vi "G#Debugger_Init.vi"(0 "This VI":refnum<vi>, 5 "error in (no error)":errorcluster) -> (14 "refs":T1, 16 "GUI Event Registration Refnum":refnum<event-registration>, 17 "Application Instance":string, 19 "error out":errorcluster)   [LabVIEW 2017, in "G#Debugger.lvlib"]
uses:
  G#Debugger.lvlib
  G#Debugger_Refs.ctl
  G#Object/utils/G#Object_ClassInfoType.ctl
  G#Object/G#Object.lvclass
  G#Object/utils/G#Object_ObjectInfoType.ctl
  G#Object/utils/G#Object_CreateMethod.ctl
  G#Debugger_SubPanelInfo.ctl
  G#Object/utils/G#Object_ClassHierarchy.ctl
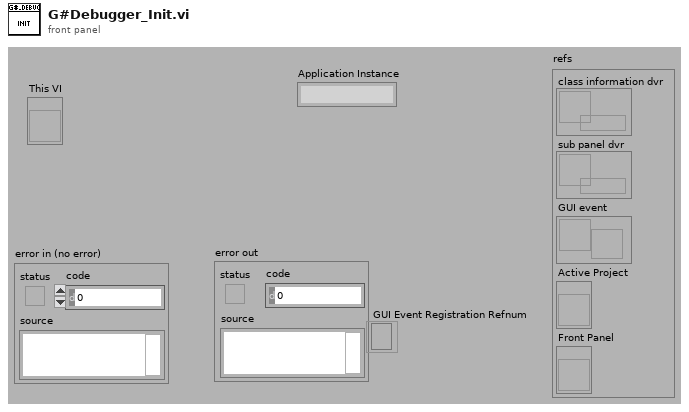
[diagram p1: front panel]
types:
  T1 = typedef "G#Debugger.lvlib/G#Debugger_Refs.ctl" = cluster{"class information dvr":refnum<data-value>, "sub panel dvr":refnum<data-value>, "GUI event":refnum<user-event>, "Active Project":refnum<vi>, "Front Panel":refnum<vi>}
  T2 = typedef "G#Debugger.lvlib/G#Debugger_SubPanelInfo.ctl" = cluster{"Ref":refnum<class "G#Object.lvclass">, "class hierarchy":T3[], "class attributes":path[], "object attributes":path[], "inheritance index":i32, "is class attributes":bool, "vi reference":refnum<vi>}
  T3 = typedef "G#Object.lvclass/G#Object_ClassHierarchy.ctl" = cluster{"ClassName":string, "FullClassName":string, "ClassPath":path, "IsLeaf":bool}
  T4 = typedef "G#Object.lvclass/G#Object_ClassInfoType.ctl" = cluster{"ClassName":string, "ObjectInfo":T5[], "ObjectRefs":refnum<class "G#Object.lvclass">[], "TypeRef":refnum<class "G#Object.lvclass">}
  T5 = typedef "G#Object.lvclass/G#Object_ObjectInfoType.ctl" = cluster{"ObjectName":string, "ObjectID":u32, "Users":i32, "Counter":bool, "AttributeRefs":u32[], "FullClassName":string, "ClassName":string, "CreateMethod":T6, "GenericDestructorExists":bool, "Owner":string}
  T6 = typedef "G#Object.lvclass/G#Object_CreateMethod.ctl" = enum16{"Create", "Create or look up existing", "Look up existing"}
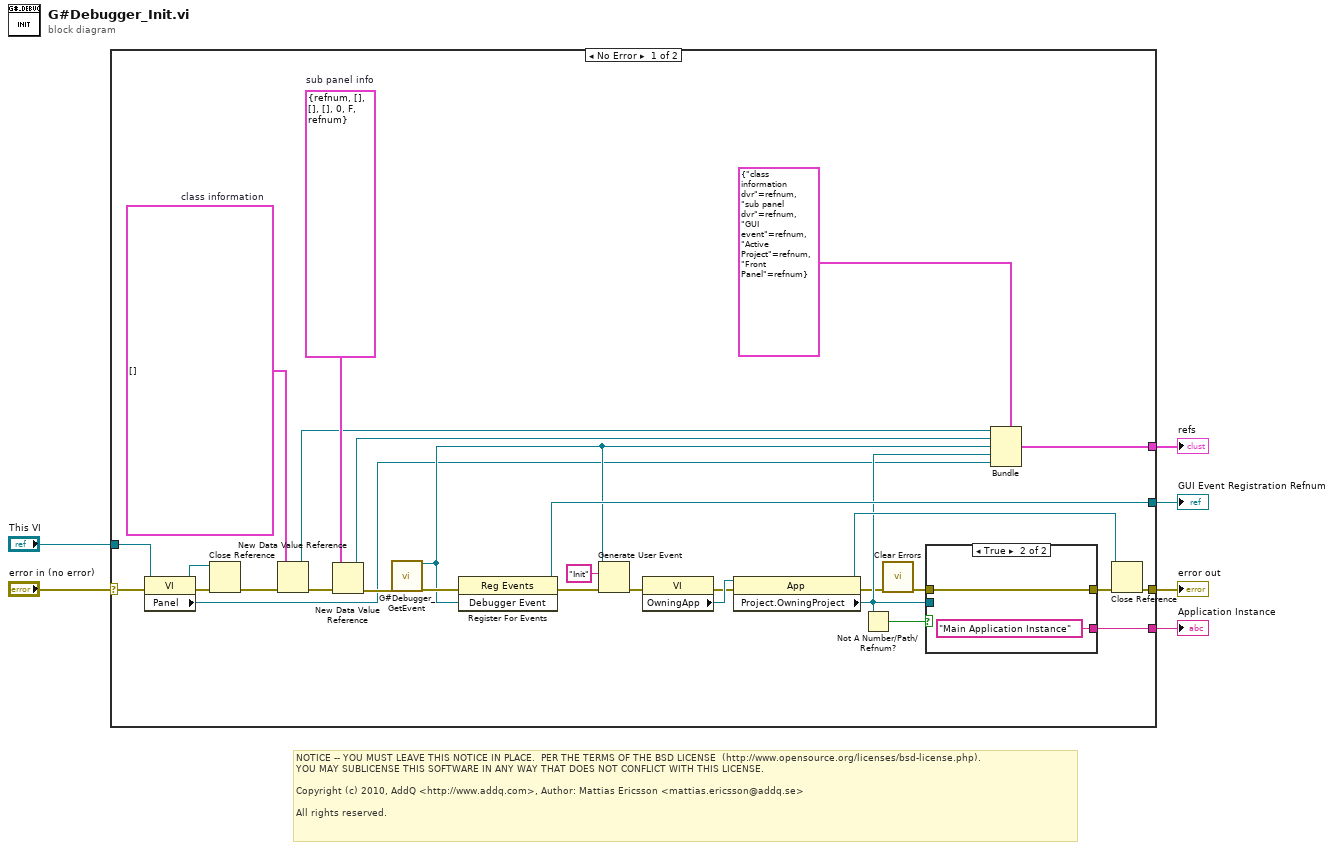
[diagram p0: block diagram]
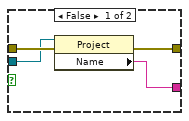
[diagram p2: hidden frame]
diagram:
  # "NOTICE -- YOU MUST LEAVE THIS NOTICE IN PLACE.  PER THE TERMS OF THE BSD LICENSE  (http://www.opensource.org/licenses/bsd-license.php).\nYOU MAY SUBLICENSE THIS SOFTWARE IN ANY WAY THAT DOES NOT CONFLICT WITH THIS LICENSE.\n\nCopyright (c) 2010, AddQ <http://www.addq.com>, Author: Mattias Ericsson <mattias.ericsson@addq.se>\n\nAll rights reserved."
  n1 = case shown="No Error" "error in (no error)" {
    selector: "error in (no error)" -> [w12 w43]
    tunnel: [w20 w43] -> w5
    tunnel: [w30 _] -> w4
    tunnel: [w27 _] -> w3
    tunnel: [w22 _] -> w2
    tunnel: "This VI" -> [w11 _]
    frame No Error {
      w33 = T2 {"Ref"=refnum, "class hierarchy"=[], "class attributes"=[], "object attributes"=[], "inheritance index"=0, "is class attributes"=FALSE, "vi reference"=refnum}  # sub panel info
      w35 = T4[] []  # class information
      n2 = property class="VI"(reference=w11, error in=w12) -> (reference out=w9:refnum<vi>, error out=w10:errorcluster, "Panel"=w8:refnum<vi>)
      n3 = Close Reference(reference=w9, error in (no error)=w10) -> (error out=w7:errorcluster)
      n4 = New Data Value Reference(data value=w35, error in=w7) -> (data value reference=w32:refnum<data-value>, error out=w34:errorcluster)
      n5 = New Data Value Reference(data value=w33, error in=w34) -> (data value reference=w31:refnum<data-value>, error out=w17:errorcluster)
      n6 = call "G#Debugger_GetEvent.vi"("error in (no error)"=w17) -> ("Debugger Event"=w15:refnum<user-event>, "error out"=w16:errorcluster)  [unwired: 17 in]
      n7 = register-events(error in=w16, w15) -> (reference out=w27:refnum<event-registration>, error out=w28:errorcluster)  [unwired: 1 in]
      n8 = Generate User Event(user event=w15, event data cluster="Init" ("event data"), error in=w28) -> (error out=w25:errorcluster)  [unwired: 1 in, 1 out]
      n9 = property class="VI"(error in=w25) -> (error out=w24:errorcluster, "OwningApp"=w26:refnum<vi>)  [unwired: 1 in, 1 out]
      n10 = property class="App"(reference=w26, error in=w24) -> (reference out=w19:refnum<vi>, error out=w14:errorcluster, "Project.OwningProject"=w18:refnum<vi>)
      n11 = Not A Number/Path/Refnum?(number/path/refnum=w18) -> (NaN/Path/Refnum?=w23:bool)
      n12 = call <vilib>:"Clear Errors.vi"("error in (no error)"=w14) -> ("error out"=w13:errorcluster)  [unwired: 5 in, 1 out]
      n13 = case shown="True" w23 {
        tunnel: w13 -> [w40 w42]
        tunnel: w18 -> [w39 _]
        tunnel: [w37 w42] -> w21
        tunnel: [w38 "Main Application Instance" ("Name")] -> w22
        frame False {
          n14 = property class="Project"(reference=w39, error in=w40) -> (error out=w37:errorcluster, "Name"=w38:string)  [unwired: 1 out]
        }
        frame True {
        }
      }
      n15 = Bundle(cluster=T1 {"class information dvr"=refnum, "sub panel dvr"=refnum, "GUI event"=refnum, "Active Project"=refnum, "Front Panel"=refnum} ("refs"), "class information dvr"=w32, "sub panel dvr"=w31, "GUI event"=w15, "Active Project"=w18, "Front Panel"=w8) -> (w30:T1)
      n16 = Close Reference(reference=w19, error in (no error)=w21) -> (error out=w20:errorcluster)
    }
    frame Error {
    }
  }
  "error out" <- w5
  "refs" <- w4
  "GUI Event Registration Refnum" <- w3
  "Application Instance" <- w2
